vi "Recurse.vi"(7 "Actor in":refnum<class "Actor.lvclass">, 8 "Error in":errorcluster, 10 "Msg":refnum<class "Msg.lvclass">) -> (0 "Error out":errorcluster, 2 "Msg Output":refnum<class "Msg Output.lvclass">, 5 "Actor out":refnum<class "Actor.lvclass">)   [LabVIEW 2020, in "jettl.lvlib"]
uses:
  jettl.lvlib
  Actor/Actor.lvclass
  Msg/Msg.lvclass
  Msg Output/Msg Output.lvclass
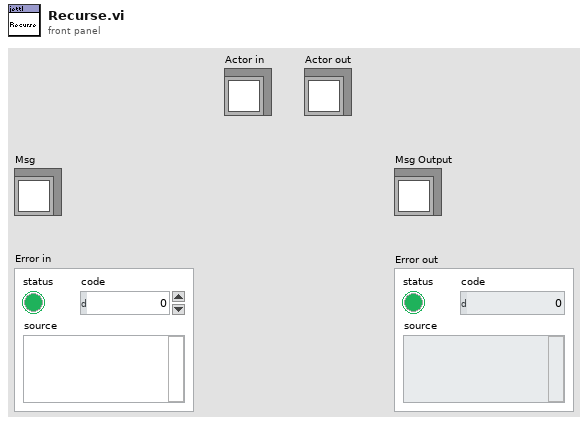
[diagram p1: front panel]
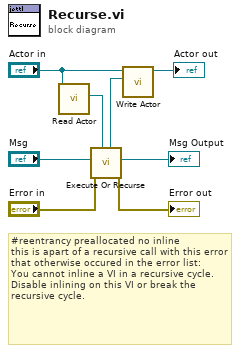
[diagram p0: block diagram]
diagram:
  # "#reentrancy preallocated no inline\nthis is apart of a recursive call with this error that otherwise occured in the error list:\nYou cannot inline a VI in a recursive cycle. Disable inlining on this VI or break the recursive cycle."
  n1 = call-dynamic "Read Actor.vi"("Actor in"="Actor in") -> ("Actor"=w4:refnum<class "Actor.lvclass">)  [unwired: 10 in]
  n2 = call "Execute Or Recurse.vi"("Actor in"=w4, "Error in"="Error in", "Msg"="Msg") -> ("Error out"=→"Error out":errorcluster, "Msg Output"=→"Msg Output":refnum<class "Msg Output.lvclass">, "Actor out"=w5:refnum<class "Actor.lvclass">)  [unwired: 6 in]
  n3 = call-dynamic "Write Actor.vi"("Actor"=w5, "Actor in"="Actor in") -> ("Actor out"=→"Actor out":refnum<class "Actor.lvclass">)  [unwired: 9 in]
